vi "Conv1D_Top.vi"() -> ()   [LabVIEW 2020]
doc: "This benchmark is designed to demonstrate execution performance improvement when executing FFT and IFFT operations on a GPU."
uses:
  <vilib>/Utility/file.llb/Read Delimited Spreadsheet (DBL).vi
  <vilib>/Analysis/1siggen.llb/Ramp Pattern by Delta.vi
  <vilib>/Ngene/CuLab - GPU Accelerated Toolkit/Toolkit/CuLab.lvlib
  <vilib>/Analysis/NI_AALBase.lvlib
panel:
  in  "CPU Iteration":i32=3
  out "CuLab Mean Performance Gain":dbl[](array[numeric])=[1.0, 21.15550240134334, 2.150127019247679] format="%#.2g"
  out "Releative Exec Time vs CuLab":cluster{i32[], "all rows":dbl[]}[](graph)=[{[32, 64, 128, 256, 512, 1024, 2048, 4096, 8192, 16384, 32768, 65536, 131072, 262144, 524288, 1048576, 2097152, 4194304, 8388608], "all rows"=[1.0, 1.0, 1.0, 1.0, 1.0, 1.0, 1.0, 1.0, 1.0, 1.0, 1.0, 1.0, 1.0, 1.0, 1.0, 1.0, 1.0, 1.0, 1.0]}, {[32, 64, 128, 256, 512, 1024, 2048, 4096, 8192, 16384, 32768, 65536, 131072, 262144, 524288, 1048576, 2097152, 4194304, 8388608], "all rows"=[0.01756007317582555, 0.016584334182935315, 0.025495751584069883, 0.046109510605750074, 0.08436639174537595, 0.19503816763949391, 0.3126022890031592, 0.6247258769756535, 1.2544094062732074, 2.7816419531963863, 5.753390257987012, 14.351283238045562, 23.17681161598989, 30.63054892919567, 40.34997783118421, 48.787817534178686, 69.9424732892676, 78.75487582579176, 84.84883334950125]}, {[32, 64, 128, 256, 512, 1024, 2048, 4096, 8192, 16384, 32768, 65536, 131072, 262144, 524288, 1048576, 2097152, 4194304, 8388608], "all rows"=[3.0383549015381206, 2.44248411598812, 2.3905807341105567, 2.454250719420757, 2.346763090589481, 3.2312977152776625, 2.3404255246144743, 2.2494517533354674, 2.2247461202747876, 2.454389959580728, 2.187845304768891, 2.112282311398667, 1.8762681175877451, 1.8483293557616274, 1.525262224523902, 1.4566653830991367, 1.5601556676397683, 1.5581714895677652, 1.554688876628257]}]
  in  "CuPy CSV":path=path "D:/Ngene/GitHub/culab_examples/Benchmarks/CuPy/results/GeForce_RTX_2080_Ti/Conv1D_CuPy.csv"
  out "Execution Time":cluster{i32[], "all rows":dbl[]}[](graph)=[{[32, 64, 128, 256, 512, 1024, 2048, 4096, 8192, 16384, 32768, 65536, 131072, 262144, 524288, 1048576, 2097152, 4194304, 8388608], "all rows"=[0.00010819999988598283, 0.00014170000031299423, 0.00014120000014372636, 0.0001388000000588363, 0.00014519999967887998, 0.00013099999978294363, 0.0001833000005717622, 0.0001824000000851811, 0.00018710000040300656, 0.0001754000004439149, 0.00019909999991796212, 0.0002181999998356332, 0.00027599999975791434, 0.00041899999996530823, 0.0006769000001440872, 0.001558800000566407, 0.0024154000002454268, 0.0048760999998194166, 0.009647300000324321]}, {[32, 64, 128, 256, 512, 1024, 2048, 4096, 8192, 16384, 32768, 65536, 131072, 262144, 524288, 1048576, 2097152, 4194304, 8388608], "all rows"=[1.8999999156221747e-06, 2.350000158912735e-06, 3.600000127335079e-06, 6.4000000747910235e-06, 1.2250000054336851e-05, 2.5549999918439426e-05, 5.729999975301325e-05, 0.00011395000001357403, 0.00023470000041925232, 0.0004878999998254585, 0.001145499999893218, 0.0031314500001826673, 0.006396800000402436, 0.012834200000270357, 0.027312899999742513, 0.0760504499999115, 0.1689390500000627, 0.38401664999992136, 0.8185621500001616]}, {[32, 64, 128, 256, 512, 1024, 2048, 4096, 8192, 16384, 32768, 65536, 131072, 262144, 524288, 1048576, 2097152, 4194304, 8388608], "all rows"=[0.00032875000000000005, 0.0003461, 0.00033755000000000005, 0.00034065000000000007, 0.00034075, 0.00042330000000000004, 0.000429, 0.0004103, 0.00041625000000000006, 0.0004305, 0.0004356, 0.00046090000000000004, 0.00051785, 0.0007744500000000001, 0.00103245, 0.00227065, 0.0037684000000000003, 0.0075978, 0.014998550000000001]}]
  out "GPU Model":string="NVIDIA GeForce RTX 2080 Ti"
  out "CPU Model":string="Intel(R) Core(TM) i7-8700K"
  in  "GPU Iteration":i32=200
  in  "Size Stop(2^n)":i32=23
  in  "Size Start(2^n)":i32=5
  out "Size":i32[](array[numeric])=[32, 64, 128, 256, 512, 1024, 2048, 4096, 8192, 16384, 32768, 65536, 131072, 262144, 524288, 1048576, 2097152, 4194304, 8388608] format="%.2p"
  # "Conv1D Benchmark"
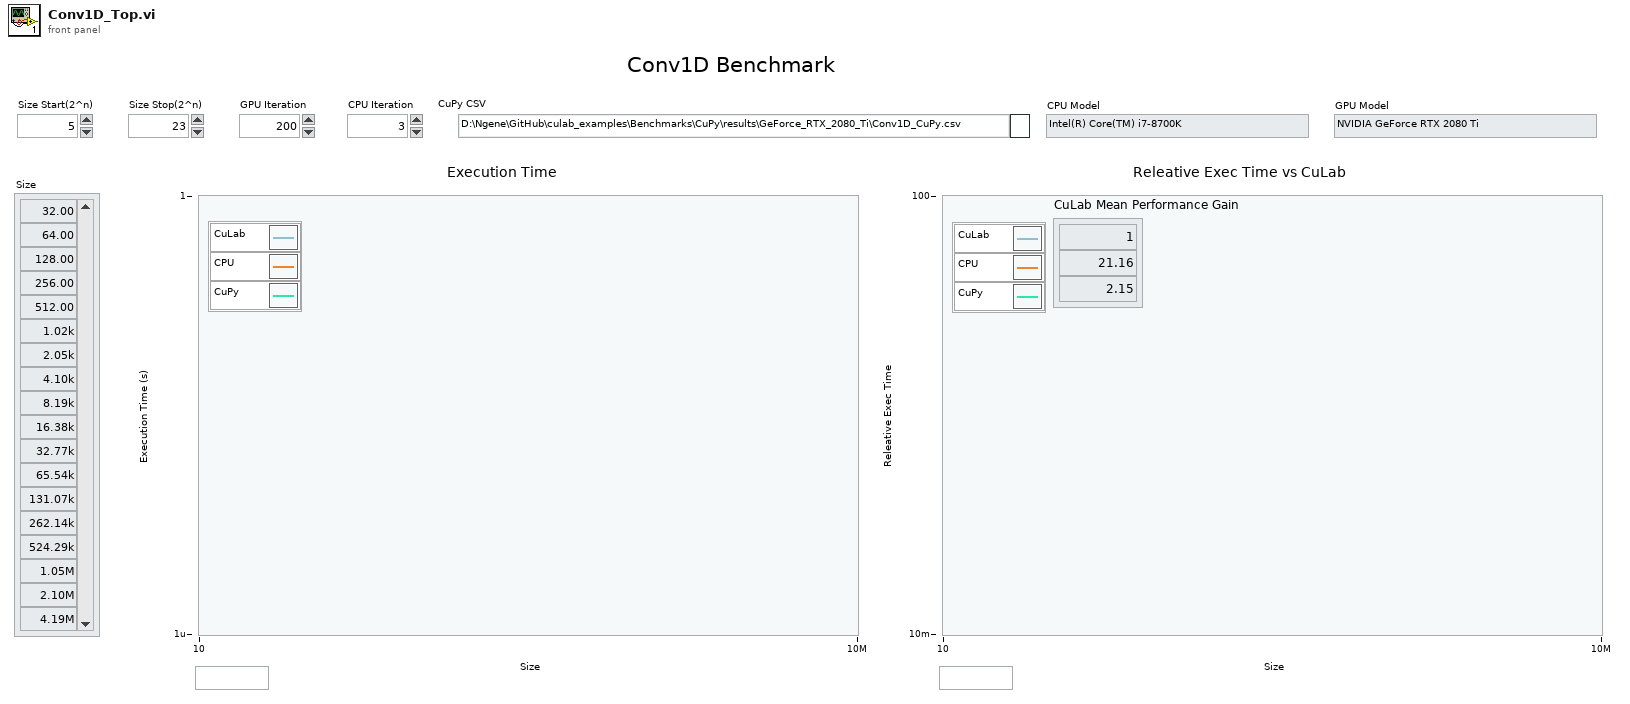
[diagram p1: front panel]
types:
  T1 = typedef "CuLab.lvlib/Properties.ctl" = cluster{"Device ID":i32, "Name":string}
  T2 = typedef "imagedata.ctl" = cluster{"image type":i32, "image depth":i32, "image":u8[], "mask":u8[], "colors":u32[], "Rectangle":cluster{"left":i16, "top":i16, "right":i16, "bottom":i16}}
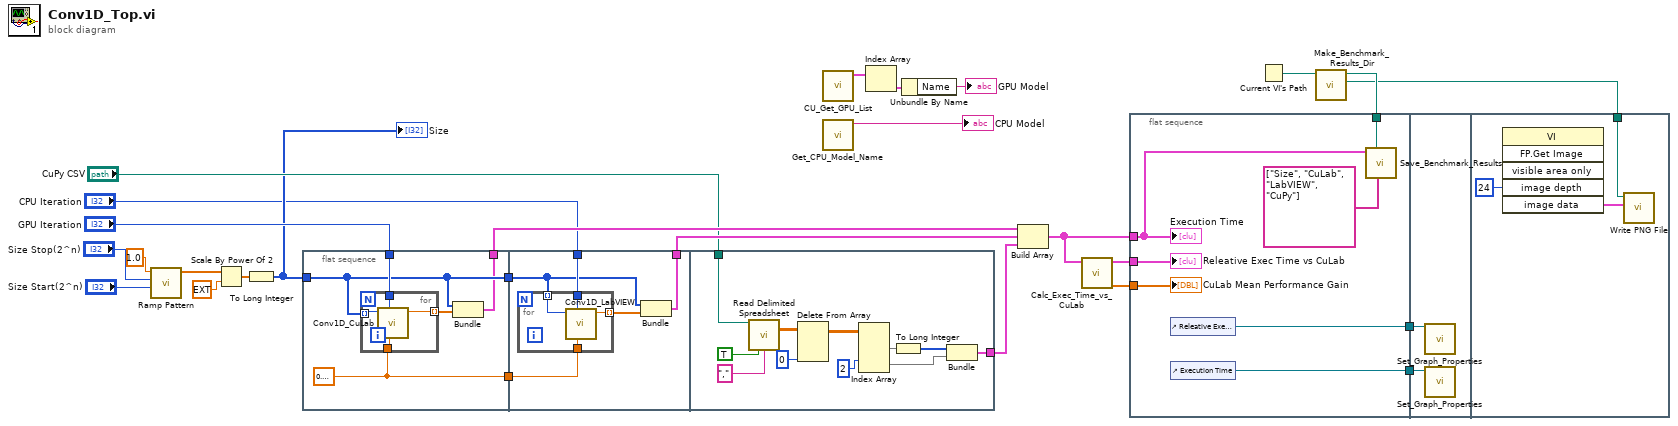
[diagram p0: block diagram]
diagram:
  n1 = call-poly <vilib>:"Ramp Pattern.vi"("start"="Size Start(2^n)", "end"="Size Stop(2^n)", "delta"=1.0) -> ("Ramp Pattern"=w13:dbl[])  [unwired: 6 in, 2 out]
  n2 = Scale By Power Of 2(n=w13, x=ext 1.0) -> (x*2^n=w15:ext[])
  n3 = To Long Integer(number=w15) -> (32bit integer=w12:i32[])
  "Size" <- w12
  n4 = flat-sequence {
    tunnel: [w29] -> w23
    tunnel: [w30] -> w24
    tunnel: w12 -> [w30]
    tunnel: "GPU Iteration" -> [w32]
    tunnel: [w28] -> w11
    tunnel: w24 -> [w39]
    tunnel: "CPU Iteration" -> [w41]
    tunnel: [w38] -> w21
    tunnel: w11 -> [w37]
    tunnel: "CuPy CSV" -> [w56]
    tunnel: [w48] -> w19
    frame #0 {
      w28 = sgl 0.1 ("Kernel Relative Size")
      n5 = for {
        tunnel: w32 -> [w35]
        tunnel: w30 -> [w36] mode=indexing
        tunnel: [w33] -> w31 mode=indexing
        tunnel: w28 -> [w34]
        n6 = call "Conv1D_CuLab.vi"("Kernel Relative Size"=w34, "No. of Repetition"=w35, "Size"=w36) -> ("Results(s)"=w33:dbl)  [unwired: 8 in]
      }
      n7 = Bundle(w30, w31) -> (w29:cluster{i32[], dbl[]})  [unwired: 1 in]
    }
    frame #1 {
      n8 = for {
        tunnel: w39 -> [w45] mode=indexing
        tunnel: w41 -> [w42]
        tunnel: [w44] -> w40 mode=indexing
        tunnel: w37 -> [w43]
        n9 = call "Conv1D_LabVIEW.vi"("Kernel Relative Size"=w43, "No. of Repetition"=w42, "Size"=w45) -> ("Results(s)"=w44:dbl)  [unwired: 8 in]
      }
      n10 = Bundle(w39, w40) -> (w38:cluster{i32[], dbl[]})  [unwired: 1 in]
    }
    frame #2 {
      n11 = call-poly <vilib>:"Read Delimited Spreadsheet.vi"("file path (dialog if empty)"=w56, "transpose? (F)"=TRUE, "delimiter (\\t)"="," ("delimiter (\\t)")) -> ("all rows"=w54:dbl[][])  [unwired: 7 in, 5 out]
      n12 = Delete From Array(array=w54, index (col)=0 ("disabled index (col)")) -> (array with subset deleted=w52:dbl[][])  [unwired: 2 in, 1 out]
      n13 = Index Array(array=w52, index (row) #2=2 ("disabled index (col)")) -> (element #1=w51:dbl[], element #2=w49:dbl[])  [unwired: 3 in]
      n14 = To Long Integer(number=w51) -> (32bit integer=w50:i32[])
      n15 = Bundle(w50, "all rows"=w49) -> (w48:cluster{i32[], "all rows":dbl[]})  [unwired: 1 in]
    }
  }
  n16 = call <vilib>:"CU_Get_GPU_List.vi"() -> ("Devices"=w26:T1[])  [unwired: 10 in, 1 out]
  n17 = call "Get_CPU_Model_Name.vi"() -> ("CPU Model"=→"CPU Model":string)  [unwired: 11 in]
  n18 = Index Array(array=w26) -> (element=w25:T1)  [unwired: 1 in]
  n19 = Unbundle By Name(w25) -> ("Name"=→"GPU Model":string)
  n20 = Build Array(w23, w21, w19) -> (w3:cluster{i32[], "all rows":dbl[]}[])
  n21 = call "Calc_Exec_Time_vs_CuLab.vi"("Exec Times"=w3) -> ("Mean Gain"=w1:dbl[], "CuLab Gain"=w2:cluster{"Array":i32[], "all rows":dbl[]}[])  [unwired: 9 in]
  n22 = flat-sequence {
    tunnel: w2 -> [w63]
    tunnel: w1 -> [w62]
    tunnel: w3 -> [w59]
    tunnel: w7 -> [w60]
    tunnel: [w58] -> w5
    tunnel: [w57] -> w4
    tunnel: w5 -> [w65]
    tunnel: w4 -> [w64]
    tunnel: w6 -> [w67]
    frame #0 {
      n23 = control-ref of="Releative Exec Time vs CuLab"() -> (w58:refnum<vi>)
      n24 = control-ref of="Execution Time"() -> (w57:refnum<vi>)
      n25 = call "Save_Benchmark_Results.vi"("Header"=string[] ["Size", "CuLab", "LabVIEW", "CuPy"], "file path (dialog if empty)"=w60, "Execution Time"=w59) -> ()  [unwired: 9 in]
      "Execution Time" <- w59
      "CuLab Mean Performance Gain" <- w62
      "Releative Exec Time vs CuLab" <- w63
    }
    frame #1 {
      n26 = call "Set_Graph_Properties.vi"("Graph"=w65) -> ()  [unwired: 11 in]
      n27 = call "Set_Graph_Properties.vi"("Graph"=w64) -> ()  [unwired: 11 in]
    }
    frame #2 {
      n28 = invoke class="VI" method="FP.Get Image"("image depth"=24 ("Image Depth")) -> ("image data"=w68:T2)  [unwired: 5 in, 5 out]
      n29 = call <vilib>:"Write PNG File.vi"("image data"=w68, "path to PNG file"=w67) -> ()  [unwired: 8 in, 2 out]
    }
  }
  n30 = Current VI's Path() -> (path=w8:path)
  n31 = call "Make_Benchmark_Results_Dir.vi"("Caller Path"=w8) -> ("Caller FP Image Path"=w6:path, "CSV_File"=w7:path)  [unwired: 9 in]
